vi "FuncVI-FileLoad.vi"(5 "InstanceRef":T2, 9 "arg list":T1[](array[typedef]) {"num" format="%.2f"}) -> (0 "error out":bool, 3 "result":T1 {"num" format="%.2f"})   [LabVIEW 2021]
doc: "::: CalcExpress Toolkit :::\nCopyright (c) 2000-2026 Konstantin Shifershteyn. All rights reserved."
uses:
  cetypes.llb/CalcExpress Function Argument Info.ctl
  cetypes.llb/CalcExpress Instance RefNum.ctl
panel:
  in  "max arg num":i32=2
  in  "min arg num":i32=2
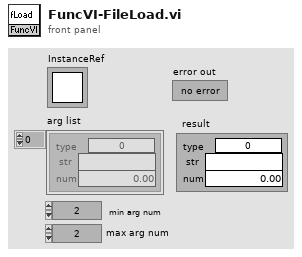
[diagram p1: front panel]
types:
  T1 = typedef "CalcExpress Function Argument Info.ctl" = cluster{"type":u32, "str":string, "num":dbl}
  T2 = typedef "CalcExpress Instance RefNum.ctl" = refnum<k1>
  T3 = cluster{"index":i32, "data type":enum32{"String", "DBL Number", "identifier", "1D Array of DBL", "2D Array of DBL", "CDB Number", "1D Array of CDB", "2D Array of CDB", "1D Array of String", "2D Array of String", "Unknown data type"}, "default num":dbl, "default str":string}[]
  T4 = enum32{"String", "DBL Number", "identifier", "1D Array of DBL", "2D Array of DBL", "CDB Number", "1D Array of CDB", "2D Array of CDB", "1D Array of String", "2D Array of String", "Unknown data type"}
  T5 = enum32{"existing file", "new file", "new or existing file", "existing dir", "new dir", "new or existing dir", "existing file (use LLBs)", "new file (use LLBs)", "new or existing file (use LLBs)", "new or existing file or directory (use LLBs)", "existing dir (use LLBs)", "new dir (use LLBs)", "new or existing dir (use LLBs)", "existing file or dir", "new file or dir", "new or existing file or dir", "existing file or dir (use LLBs)", "new file or dir (use LLBs)"}
  T6 = typedef "VarMan Variable Context Handle.ctl" = i32
  T7 = cluster{"type: use this constant to specify a predefined type code":enum32{"String", "DBL Number", "identifier", "1D Array of DBL", "2D Array of DBL", "CDB Number", "1D Array of CDB", "2D Array of CDB", "1D Array of String", "2D Array of String", "Unknown data type"}, string, dbl}
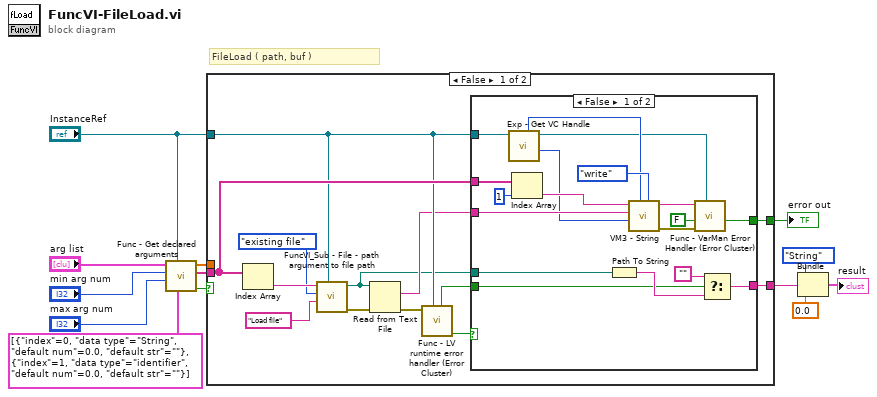
[diagram p0: block diagram]
diagram:
  # "FileLoad ( path, buf )"
  n1 = call "Func - Get declared arguments.vi"("arg descriptors"=T3 [{"index"=0, "data type"=enum."String", "default num"=0.0, "default str"=""}, {"index"=1, "data type"=enum."identifier", "default num"=0.0, "default str"=""}] ("args descriptors"), "InstanceRef"="InstanceRef", "max arg num"="max arg num", "min arg num"="min arg num", "arg list"="arg list") -> ("error out"=w8:bool, "str list"=w9:string[], "num list"=w5:dbl[])  [unwired: 3 in, 1 out]
  n2 = case shown="False" w8 {
    selector: w8 -> [_ w46]
    tunnel: "InstanceRef" -> [w20 _]
    tunnel: w9 -> [w23 _]
    tunnel: [w21 _] -> w3
    tunnel: w5 -> [_ _]
    tunnel: [w22 w46] -> w4
    frame False {
      n3 = Index Array(array=w23) -> (element=w26:string)  [unwired: 1 in]
      n4 = call "FuncVI_Sub - File - path argument to file path.vi"("InstanceRef"=w20, "prompt"="Load file", "select mode (2)"=T5."existing file", "arg: file path"=w26) -> ("error out"=w16:errorcluster, "file path"=w14:path)  [unwired: 5 in, 1 out]
      n5 = Read from Text File(file (use dialog)=w14, error in=w16) -> (text=w17:string, error out=w15:errorcluster)  [unwired: 2 in, 2 out]
      n6 = call "Func - LV runtime error handler (Error Cluster).vi"("InstanceRef"=w20, "LabVIEW error"=w15) -> ("error out"=w18:bool, "LV error status"=w19:bool)  [unwired: 4 in, 2 out]
      n7 = case shown="False" w18 {
        selector: w18 -> [_ w45]
        tunnel: w20 -> [w42 _]
        tunnel: w23 -> [w43 _]
        tunnel: [w29 w45] -> w22
        tunnel: w14 -> [w41 _]
        tunnel: w17 -> [w31 _]
        tunnel: [w39 _] -> w21
        tunnel: w19 -> [w37 _]
        frame False {
          n8 = call "Exp - Get VC Handle.vi"("InstanceRef"=w42) -> ("writer ID"=w30:u32, "dup InstanceRef"=w27:T2, "VC Handle"=w33:T6)  [unwired: 5 in, 1 out]
          n9 = Index Array(array=w43, index=1) -> (element=w32:string)
          n10 = Path To String(path=w41) -> (string=w40:string)
          n11 = call "VM3 - String.vi"("cmd (read)"=enum16{"create", "destroy", "write", "read"}."write", "VC Handle"=w33, "writer ID"=w30, "value in"=w31, "name_spec"=w32) -> ("error out"=w36:errorcluster, "dup name_spec"=w35:string)  [unwired: 3 in, 2 out]
          n12 = call "Func - VarMan Error Handler (Error Cluster).vi"("InstanceRef"=w27, "VarMan VI error in"=w36, "error status before"=FALSE, "var name"=w35) -> ("FuncVI error out"=w29:bool)  [unwired: 5 in, 2 out]
          n13 = Select(t="", s=w37, f=w40) -> (s? t:f=w39:string)
        }
        frame True {
        }
      }
    }
    frame True {
    }
  }
  "error out" <- w4
  n14 = Bundle("type: use this constant to specify a predefined type code"=T4."String", w3, 0.0) -> (→"result":T7)  [unwired: 1 in]
